vi "SetSelectedChannel.vi"(8 "error in (no error)":errorcluster, 10 "Channel Name":string, 11 "object in":refnum<class "ChannelManagerUI.lvclass">) -> (0 "error out":errorcluster, 3 "object out":refnum<class "ChannelManagerUI.lvclass">)   [LabVIEW 2021, in "Channel.lvlib" / "ChannelManagerUI.lvlib" / "ChannelManagerUI.lvclass"]
uses:
  ChannelManagerUI.lvclass
  C:/Users/averna/Documents/LV Gym DEMO/Factory Pattern/Generic Channel/ChannelsManager/ChannelsManager/ChannelsManager.lvclass
  ChannelManagerUI.lvclass/ChannelManagerUI.ctl
  Channel_class/Channel.lvclass
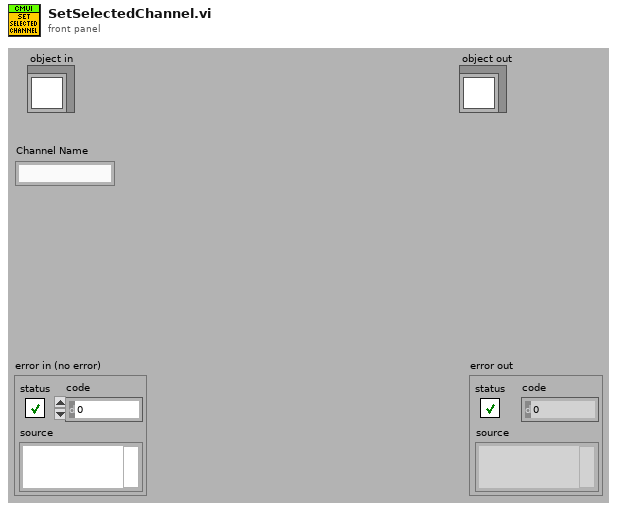
[diagram p1: front panel]
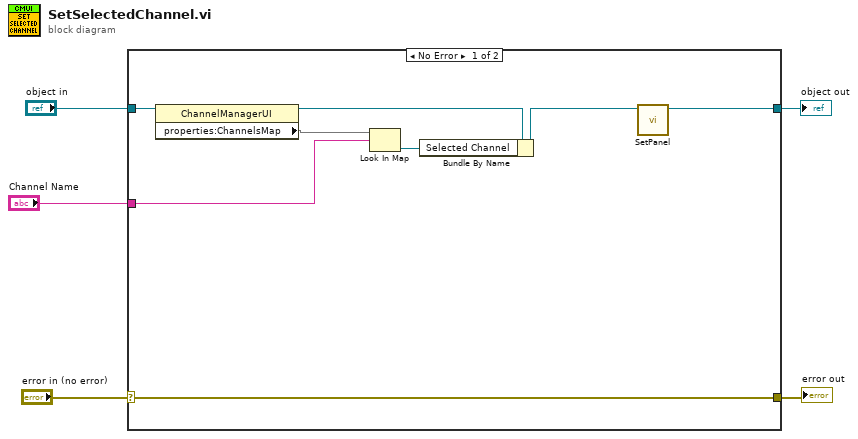
[diagram p0: block diagram]
diagram:
  n1 = case shown="No Error" "error in (no error)" {
    selector: "error in (no error)" -> [w13 w15]
    tunnel: [w13 w15] -> w4
    tunnel: [w6 w14] -> w2
    tunnel: "object in" -> [w12 w14]
    tunnel: "Channel Name" -> [w9 _]
    frame No Error {
      n2 = property class="ChannelManagerUI"(reference=w12) -> (reference out=w11:refnum<class "ChannelManagerUI.lvclass">, "properties:ChannelsMap"=w10:map{string, refnum<class "Channel.lvclass">})  [unwired: 1 in, 1 out]
      n3 = Look In Map(map=w10, key=w9) -> (value=w7:refnum<class "Channel.lvclass">)  [unwired: 1 in, 1 out]
      n4 = Bundle By Name(cluster=w11, "Selected Channel"=w7) -> (w8:refnum<class "ChannelManagerUI.lvclass">)
      n5 = call-dynamic "SetPanel.vi"("ChannelManagerUI in"=w8) -> ("ChannelManagerUI out"=w6:refnum<class "ChannelManagerUI.lvclass">)  [unwired: 9 in, 1 out]
    }
    frame Error {
    }
  }
  "error out" <- w4
  "object out" <- w2
